vi "Queue-Daily Roll-up.vi"(8 "error in":errorcluster, 10 "Data":variant, 11 "Queue In":refnum<queue>) -> (0 "error out":errorcluster, 3 "Queue Out":refnum<queue>)   [LabVIEW 2026, in "Main_Process.lvlib" / "Internal Messaging Library.lvlib"]
doc: "<B>Description:</B> Sends Data to the Daily Roll-up Case of Internal Processing for the Event Logger.\n\n<B>Date:</B> 11/2026 \n<B>Author:</B> Erich Schlieper"
uses:
  Controls/Messaging Cluster.ctl
  Controls/Message.ctl
  Internal Messaging Library.lvlib
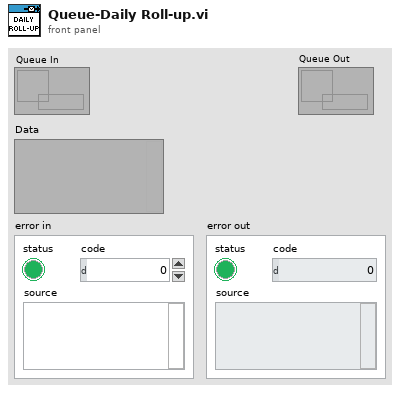
[diagram p1: front panel]
types:
  T1 = typedef "Main_Process.lvlib/Internal Messaging Library.lvlib/Message.ctl" = enum16{"Initialize", "Exit", "Error", "Load Data", "Add Project", "Edit Project", "Add Time Entry", "End Time Entry", "Save Project(s)", "Update Project List", "Inactivate Project", "Update Task List", "Inactivate Task", "Modify Time Entry", "Update Time Entry", "Delete Time Entry", "Pause Time Entry Update", "Load Data for Month", "Daily Roll-up"}
  T2 = typedef "Main_Process.lvlib/Internal Messaging Library.lvlib/Messaging Cluster.ctl" = cluster{"Message":T1, "Data":variant}
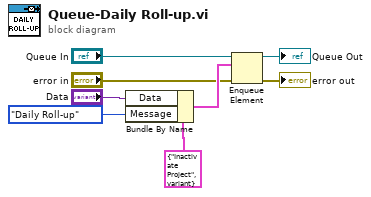
[diagram p0: block diagram]
diagram:
  n1 = Bundle By Name(cluster=T2 {"Message"=enum."Inactivate Project", "Data"=variant} ("Messaging Cluster"), "Data"="Data", "Message"=Message."Daily Roll-up") -> (w8:T2)
  n2 = Enqueue Element(queue="Queue In", element=w8, error in (no error)="error in") -> (queue out=→"Queue Out":refnum<queue>, error out=→"error out":errorcluster)  [unwired: 1 in, 1 out]
